vi "RDC-add_ideal_perm.vi"(7 "water Temp (25C) [10-40C]":dbl=25.0, 8 "Salt Water":T1, 9 "DI-Water":T1, 10 "Open/Air":T1) -> (0 "Salt Water out":T1, 1 "DI-Water  out":T1, 2 "Open/Air out":T1)   [LabVIEW 2020, in "RDC-Reflection_Data_Computation.lvlib"]
doc: "Fills in the permittivity of the three calibration standards: 1 and 0 for Open/Air, and the model values of DI water and salt water at the given water temperature (10-40 C) for their frequencies."
uses:
  RDC-Reflection_Data_Computation.lvlib
  Reflector/RFH-common_data_format.ctl
  Reflector/RFH-Reflection_File_Handler.lvlib
panel:
  out "Waveform Graph":dbl[](graph)
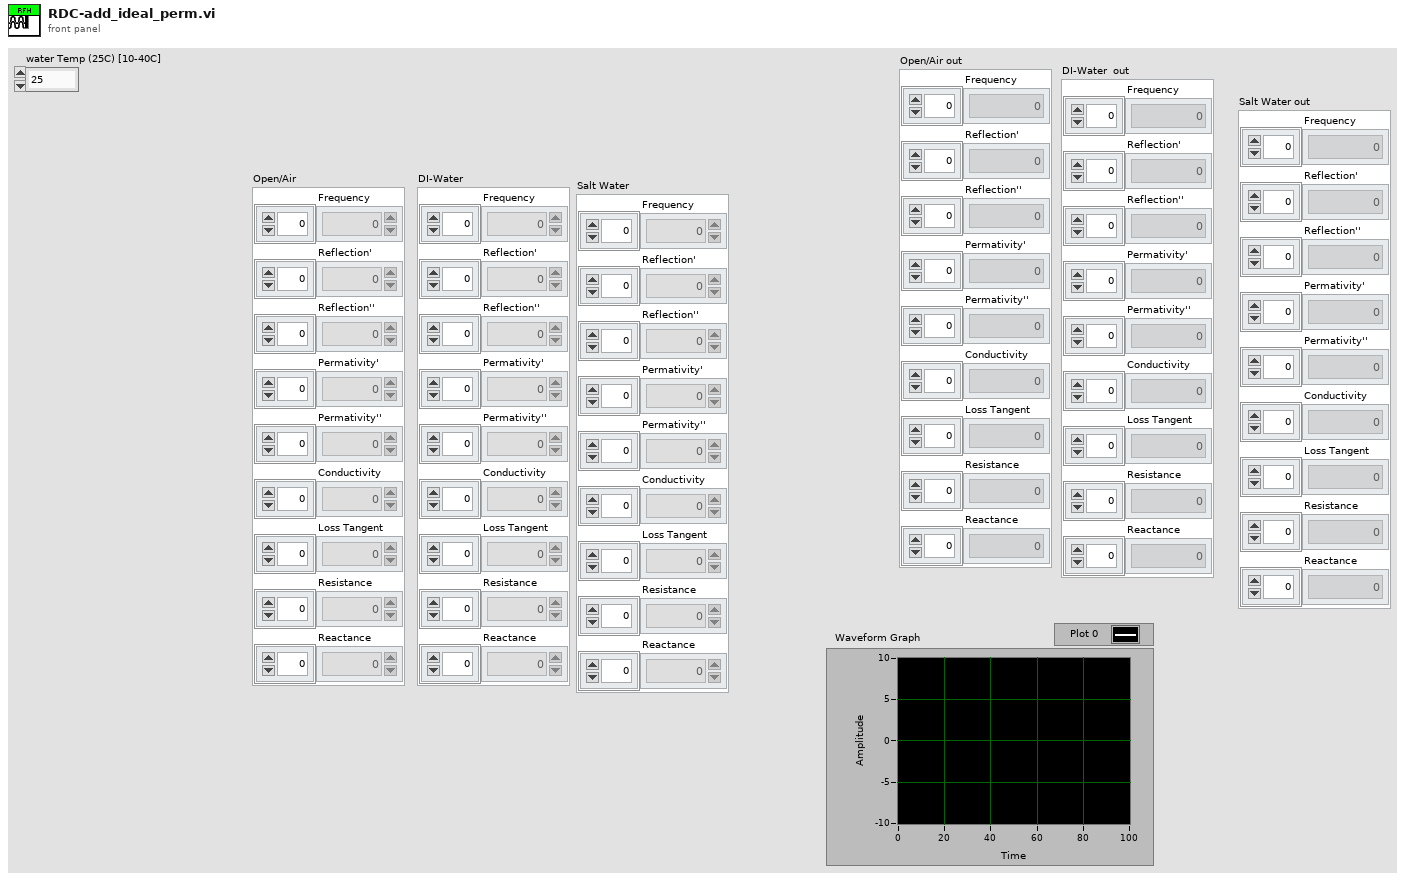
[diagram p1: front panel]
types:
  T1 = typedef "RFH-Reflection_File_Handler.lvlib/RFH-common_data_format.ctl" = cluster{"Frequency":dbl[], "Reflection'":dbl[], "Reflection''":dbl[], "Permativity'":dbl[], "Permativity''":dbl[], "Conductivity":dbl[], "Loss Tangent":dbl[], "Resistance":dbl[], "Reactance":dbl[]}
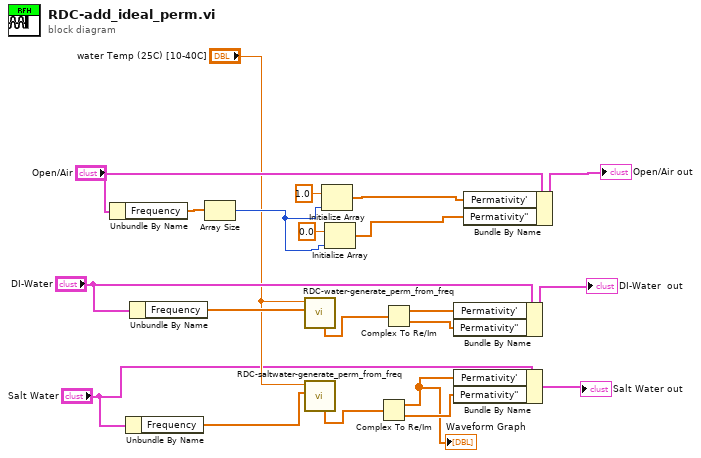
[diagram p0: block diagram]
diagram:
  n1 = Unbundle By Name("Open/Air") -> ("Frequency"=w19:dbl[])
  n2 = Unbundle By Name("Salt Water") -> ("Frequency"=w6:dbl[])
  n3 = Unbundle By Name("DI-Water") -> ("Frequency"=w13:dbl[])
  n4 = Array Size(array=w19) -> (size(s)=w18:i32)
  n5 = call "RDC-water-generate_perm_from_freq.vi"("Frequency"=w13, "water Temp (25C) [10-40C]"="water Temp (25C) [10-40C]") -> ("Complex perm"=w10:cdb[])  [unwired: 5 in, 4 out]
  n6 = call "RDC-saltwater-generate_perm_from_freq.vi"("Frequency"=w6, "water Temp (25C) [10-40C]"="water Temp (25C) [10-40C]") -> ("Complex perm"=w3:cdb[])  [unwired: 6 in, 3 out]
  n7 = Initialize Array(1.0 ("element"), w18) -> (w15:dbl[])
  n8 = Initialize Array(0.0 ("element"), w18) -> (w14:dbl[])
  n9 = Complex To Re/Im(x + iy=w3) -> (x=w1:dbl[], y=w2:dbl[])
  "Waveform Graph" <- w1
  n10 = Complex To Re/Im(x + iy=w10) -> (x=w9:dbl[], y=w8:dbl[])
  n11 = Bundle By Name(cluster="DI-Water", "Permativity'"=w9, "Permativity''"=w8) -> (→"DI-Water  out":T1)
  n12 = Bundle By Name(cluster="Salt Water", "Permativity'"=w1, "Permativity''"=w2) -> (→"Salt Water out":T1)
  n13 = Bundle By Name(cluster="Open/Air", "Permativity'"=w15, "Permativity''"=w14) -> (→"Open/Air out":T1)
